vi "test_GetItemInfosFromProjectFile_HierarchyExampleProject.vi"() -> (3 "Pass?":bool)   [LabVIEW 2019, in "Tests.SolutionBuilder.lvlib"]
uses:
  Tests.SolutionBuilder.lvlib
  SolutionBuilder/SolutionBuilder.lvclass
  SolutionBuilder/ProjectItem/ProjectItem.lvclass
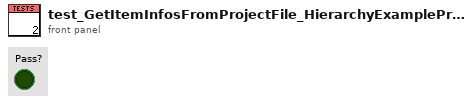
[diagram p1: front panel]
types:
  T1 = typedef "SolutionBuilder.lvlib/SolutionBuilder.lvclass/ProjectItemMap.ctl" = map{path, refnum<class "ProjectItem.lvclass">[]}
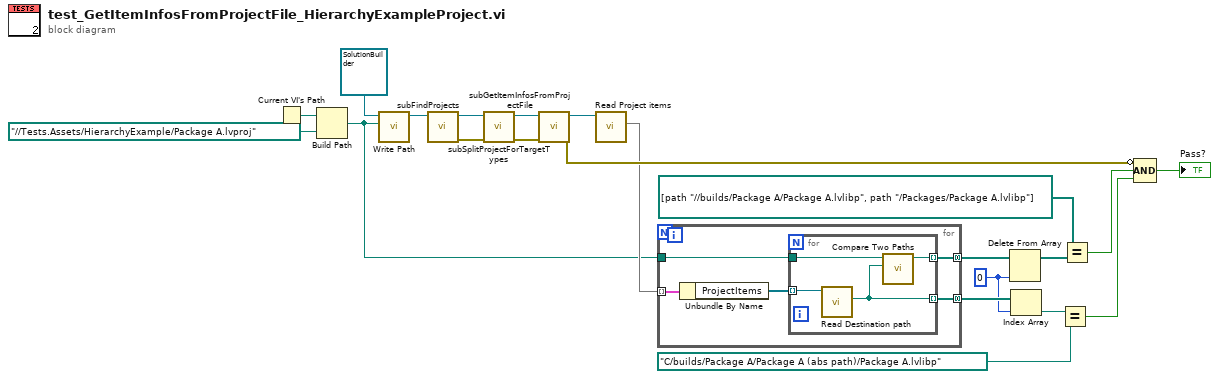
[diagram p0: block diagram]
diagram:
  w8 = 0 ("index")
  n1 = Current VI's Path() -> (path=w20:path)
  n2 = Build Path(base path=w20, name or relative path=path "../../Tests.Assets/HierarchyExample/Package A.lvproj" ("Path")) -> (appended path=w14:path)
  n3 = call "Write Path.vi"("Path"=w14, "SolutionBuilder in"=refnum<class "SolutionBuilder.lvclass"> refnum) -> ("SolutionBuilder out"=w21:refnum<class "SolutionBuilder.lvclass">)  [unwired: 9 in]
  n4 = call "subFindProjects.vi"("SolutionBuilder in"=w21) -> ("error out"=w1:errorcluster, "SolutionBuilder out"=w4:refnum<class "SolutionBuilder.lvclass">)  [unwired: 9 in]
  n5 = call "subSplitProjectForTargetTypes.vi"("error in (no error)"=w1, "SolutionBuilder in"=w4) -> ("error out"=w2:errorcluster, "SolutionBuilder out"=w3:refnum<class "SolutionBuilder.lvclass">)  [unwired: 8 in]
  n6 = call "subGetItemInfosFromProjectFile.vi"("error in (no error)"=w2, "SolutionBuilder in"=w3) -> ("error out"=w18:errorcluster, "SolutionBuilder out"=w16:refnum<class "SolutionBuilder.lvclass">)  [unwired: 8 in]
  n7 = call "Read Project items.vi"("SolutionBuilder in"=w16) -> ("Project items"=w15:T1)  [unwired: 9 in, 1 out]
  n8 = for {
    tunnel: w15 -> [w27] mode=indexing
    tunnel: [w25] -> w11 mode=concatenating
    tunnel: w14 -> [w24]
    tunnel: [w23] -> w9 mode=concatenating
    n9 = Unbundle By Name(w27) -> ("ProjectItems"=w26:refnum<class "ProjectItem.lvclass">[])
    n10 = for {
      tunnel: w26 -> [w31] mode=indexing
      tunnel: [w29] -> w25 mode=indexing
      tunnel: w24 -> [w30]
      tunnel: [w28] -> w23 mode=indexing
      n11 = call "Read Destination path.vi"("ProjectItem in"=w31) -> ("Destination path"=w28:path)  [unwired: 9 in, 1 out]
      n12 = call <vilib>:"Compare Two Paths.vi"("Path 2"=w28, "Path 1"=w30) -> ("Relative Path from 1 to 2"=w29:path)  [unwired: 6 in, 3 out]
    }
  }
  n13 = Delete From Array(array=w11, index=w8) -> (array with subset deleted=w10:path[])  [unwired: 1 in, 1 out]
  n14 = Index Array(array=w9, index=w8) -> (element=w7:path)
  n15 = Equal?(x=w7, y=path "C:/builds/Package A/Package A (abs path)/Package A.lvlibp" ("Relative Path from 1 to 2")) -> (x = y?=w5:bool)
  n16 = Equal?(x=path[] [path "../../builds/Package A/Package A.lvlibp", path "../Packages/Package A.lvlibp"] ("y"), y=w10) -> (x = y?=w12:bool)
  n17 = Compound Arithmetic op=AND(invert w18, w12, w5) -> (→"Pass?":bool)
